vi "Measurement UI.vi"() -> ()   [LabVIEW 2022 SP3, in "Single Tone No Gen_Class D Amplifier_UI.lvlib"]
uses:
  Single Tone No Gen_Class D Amplifier_UI.lvlib
  shared/controls/units - snr.ctl
  shared/controls/units - ratio.ctl
  shared/ui/controls/view.ctl
  shared/controls/acquisition type.ctl
  UI State.ctl
  <vilib>/Utility/miscctls.llb/LVBoundsTypeDef.ctl
  <vilib>/Utility/miscctls.llb/LVPoint32TypeDef.ctl
  <vilib>/Utility/miscctls.llb/LVPointTypeDef.ctl
  shared/ui/UI Helpers.lvlib
  shared/audio popup ui/Audio Popup UI.lvlib
  shared/controls/audio controls.lvlib
panel:
  in  "view legend":T1
  out "time domain":waveform(dbl)[](graph)
  out "frequency domain":cluster{"x0":dbl, "dx":dbl, "magnitude":dbl[]}[](graph)
  out "meas table":string[][](table)
  in  "input configuration file":string
  out "output power (W)":dbl[](array[numeric])
  out "SFDR (dBc)":dbl[](array[numeric])
  out "gain":dbl[](array[numeric])
  out "dynamic range (dB)":dbl[](array[numeric])
  out "THD":dbl[](array[numeric])
  out "THD+N":dbl[](array[numeric])
  out "SNR":dbl[](array[numeric])
  out "phase (deg)":dbl[](array[numeric])
  out "amplitude (dBFS)":dbl[](array[numeric])
  out "amplitude (Vrms)":dbl[](array[numeric])
  out "frequency (Hz)":dbl[](array[numeric])
  out "channel names":string[](array[string])
  in  "Configuration tab":enum32{"Acquisition", "Measurement", "Units"}(tab)
  in  "digital channel list":string caption="Digital audio channel"
  in  "configure input":bool
  in  "acquisition type":T2 caption="Input Type"
  in  "Acquisition channel":tag
  in  "min measurement time (s)":dbl=0.1 caption="Minimum measurement time" format="%#_6ps"
  in  "min measurement cycles":u32 caption="Minimum measurement cycles"
  in  "min settling time (s)":dbl=0.1 caption="Minimum settling time" format="%#_6ps"
  in  "min settling cycles":u32 caption="Minimum settling cycles"
  in  "expected amplitude (Vpk)":dbl=1000.0 caption="Expected amplitude" format="%#_6f Vpk"
  in  "lowpass filter":T3(ring) caption="Lowpass filter"
  in  "highpass filter":enum32{"DC", "AC"}(ring) caption="Highpass filter"
  in  "band start":dbl=20.0 caption="Band start" format="%#_6pHz"
  in  "band stop":dbl=20000.0 caption="Band stop" format="%#_6pHz"
  in  "weighting filter":T4(ring)=enum."A-weighting" caption="Weighting filter"
  in  "load impedance":dbl=4.0 caption="Load impedance" format="%#_6p Ohms"
  in  "amplitude reference (Vpk-pk)":dbl=15.0 caption="Amplitude reference" format="%.3p Vpk-pk"
  in  "expected signal frequency":dbl=1000.0 caption="Expected frequency" format="%#_6pHz"
  in  "gain units":T5 caption="Gain"
  in  "THD units":T5 caption="THD"
  in  "THD+N units":T5 caption="THD+N"
  in  "SNR units":T6 caption="SNR"
  out "fft - data":dbl[](array[numeric])
  out "fft - df":dbl
  out "fft - f0":dbl
  out "wfm - data":dbl[](array[numeric])
  out "wfm - dt":dbl
  out "wfm - t0":dbl
  in  "analog input channel":string="PXI1Slot4/ai0"
  # "hidden controls - used to sync with MeasLink"
  # "hidden indicators"
  # "Acquisition"
  # "Filters"
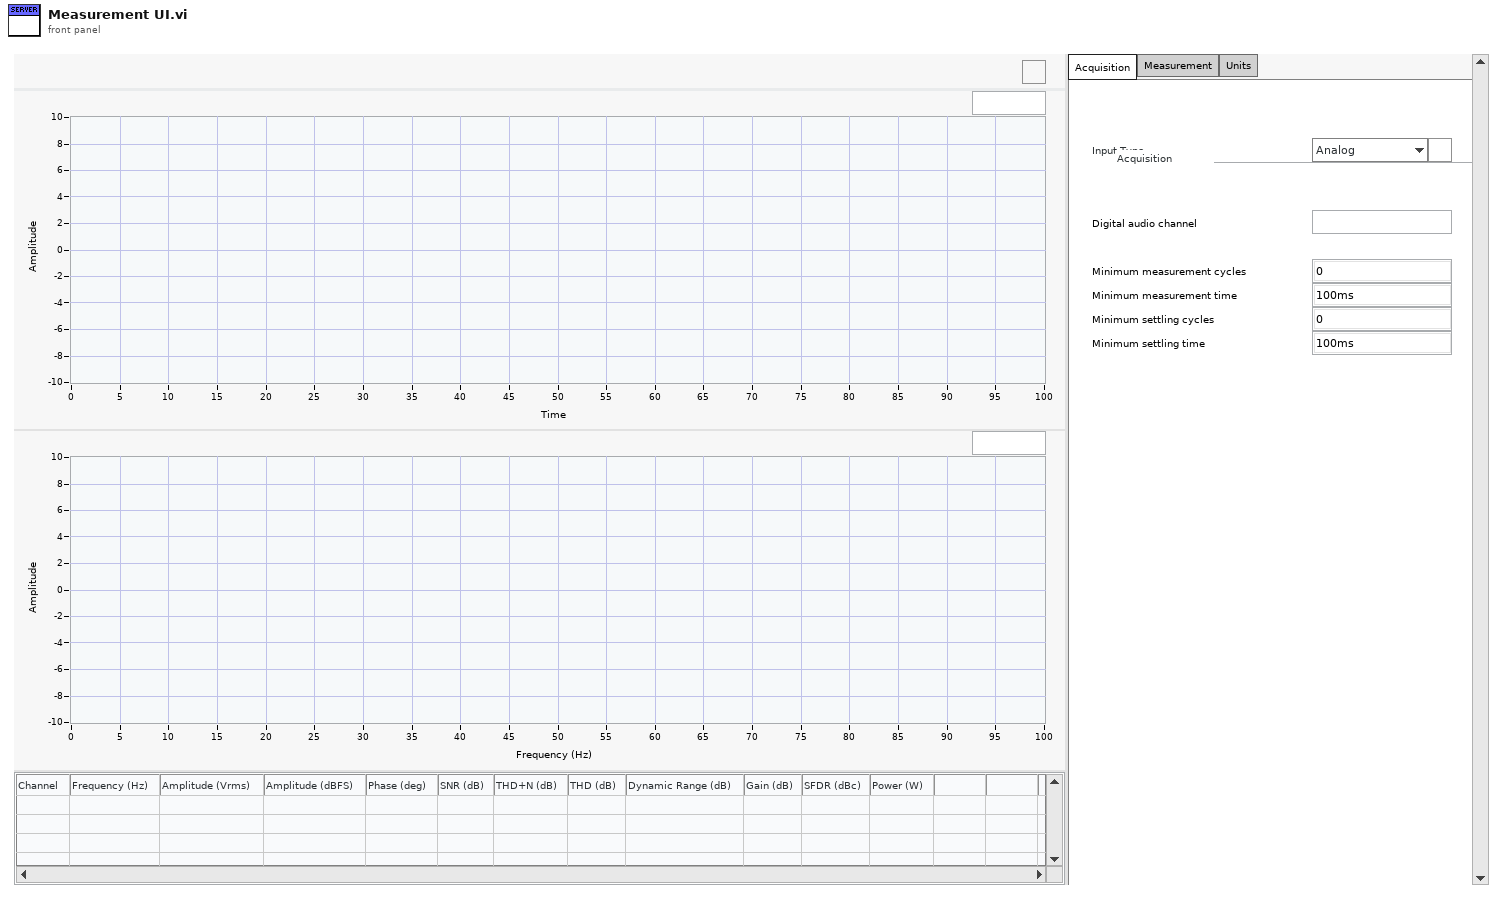
[diagram p1: front panel]
types:
  T1 = typedef "UI Helpers.lvlib/view.ctl" = bool
  T2 = typedef "acquisition type.ctl" = enum32{"Analog", "Digital Serial"}
  T3 = enum32{"No filter", "AES17 20kHz", "AES17 40kHz"}
  T4 = enum32{"Linear", "A-weighting", "B-weighting", "C-weighting"}
  T5 = typedef "audio controls.lvlib/units - ratio.ctl" = enum32{"dB", "%", "x/y"}
  T6 = typedef "audio controls.lvlib/units - snr.ctl" = enum32{"dB", "x/y"}
  T7 = typedef "Single Tone No Gen_Class D Amplifier_UI.lvlib/UI State.ctl" = cluster{"Graph Size":T8, "Legend Visible":bool, "Mouse Coords":T9, "Show All Plots":bool, "digital serial cfg file":path, "analog cfg file":path, "PostUI event occurred":bool}
  T8 = typedef "LVBoundsTypeDef.ctl" = cluster{"Width":u32, "Height":u32}
  T9 = typedef "LVPoint32TypeDef.ctl" = cluster{"Horizontal":i32, "Vertical":i32}
  T10 = typedef "LVPointTypeDef.ctl" = cluster{"Horizontal":i16, "Vertical":i16}
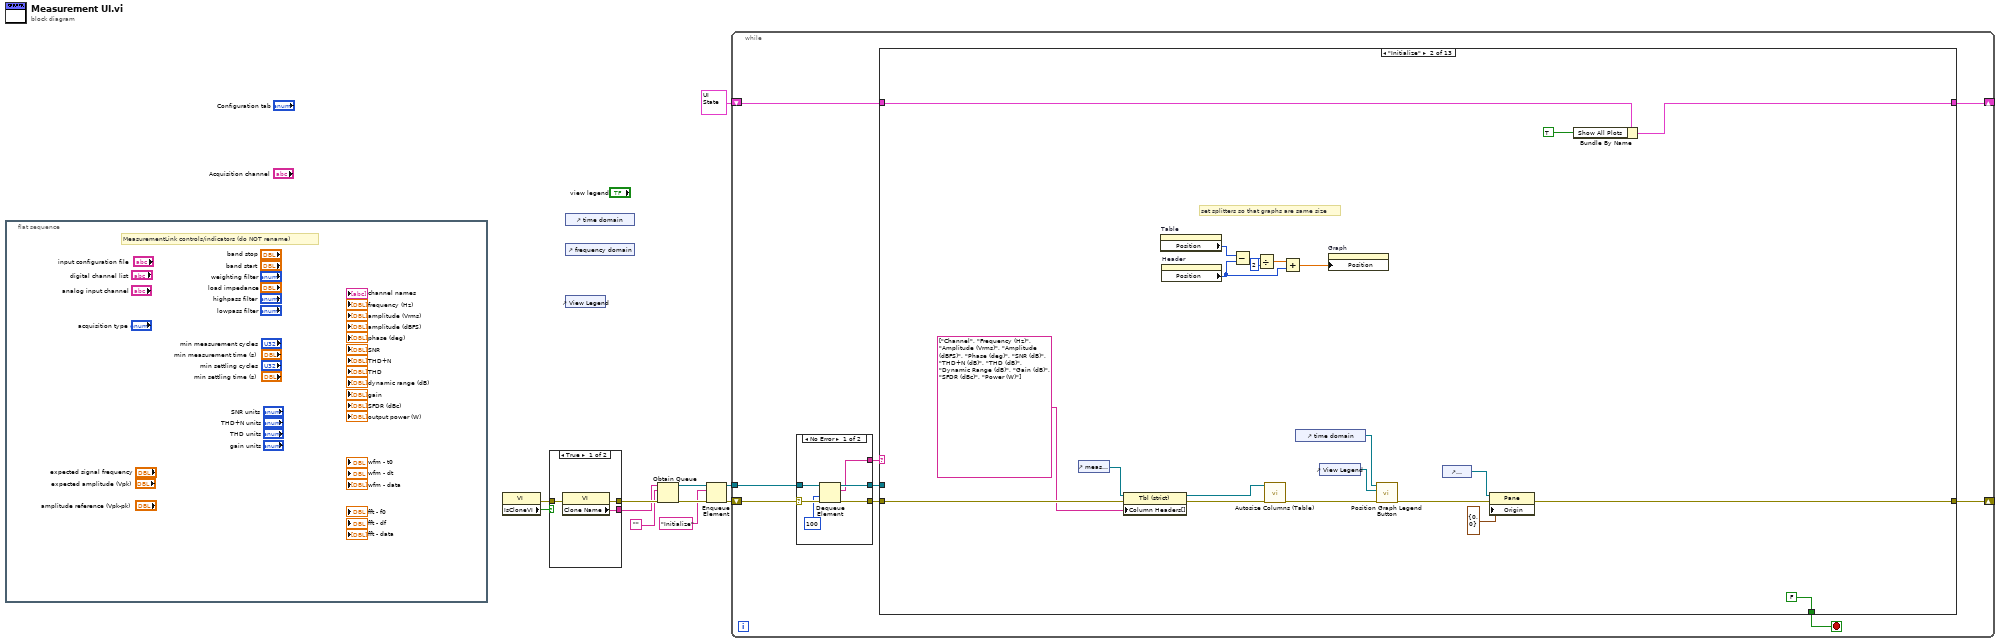
[diagram p0: block diagram]
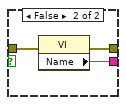
[diagram p2: hidden frame]
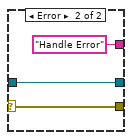
[diagram p3: hidden frame]
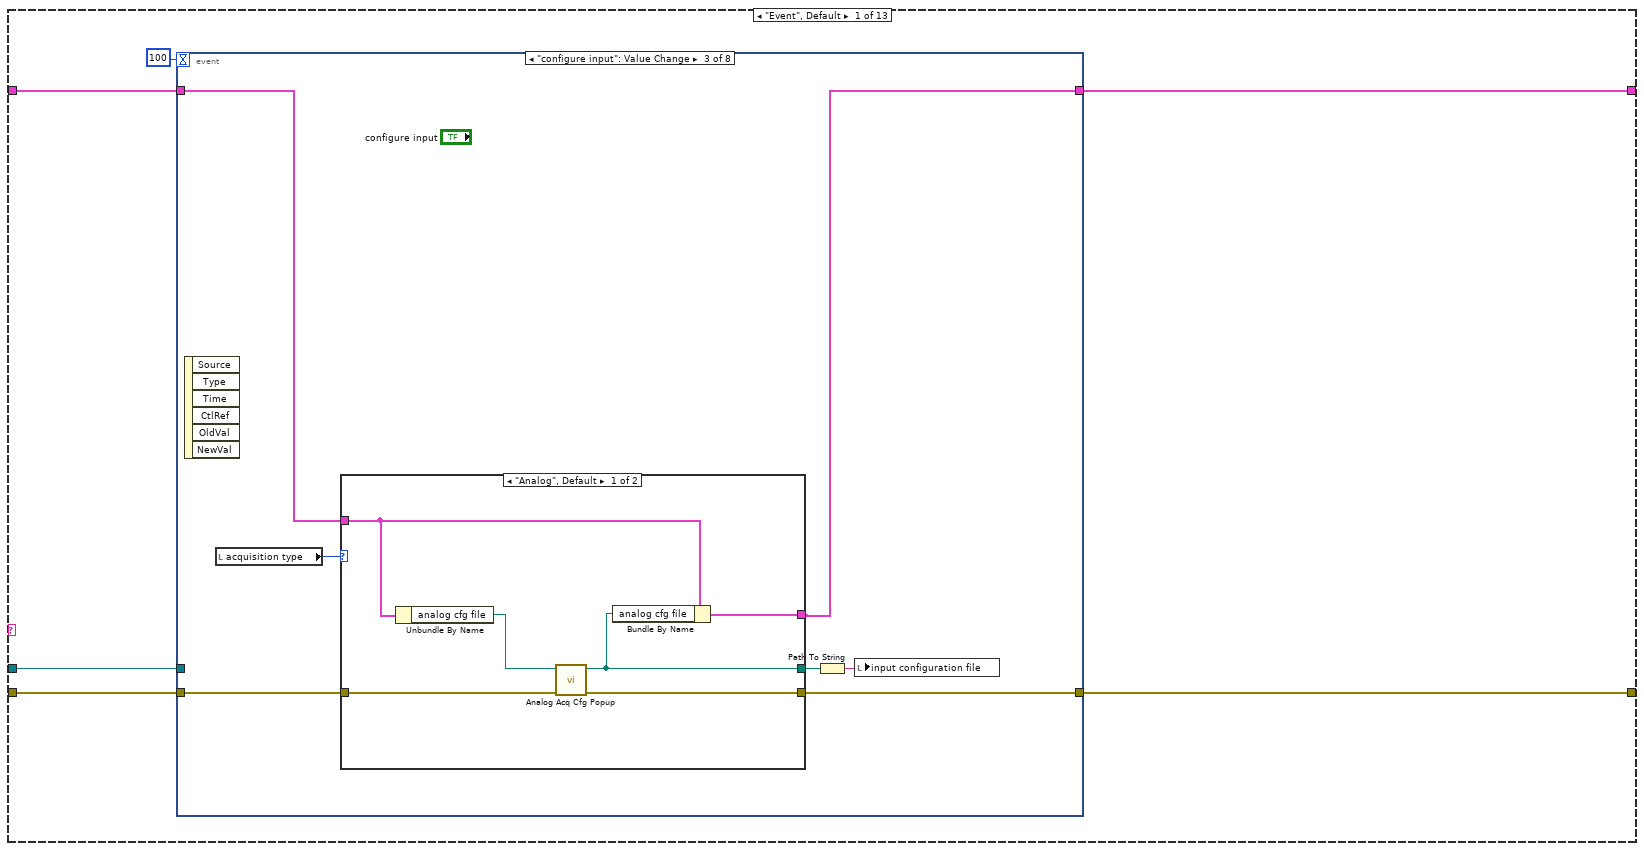
[diagram p4: hidden frame]
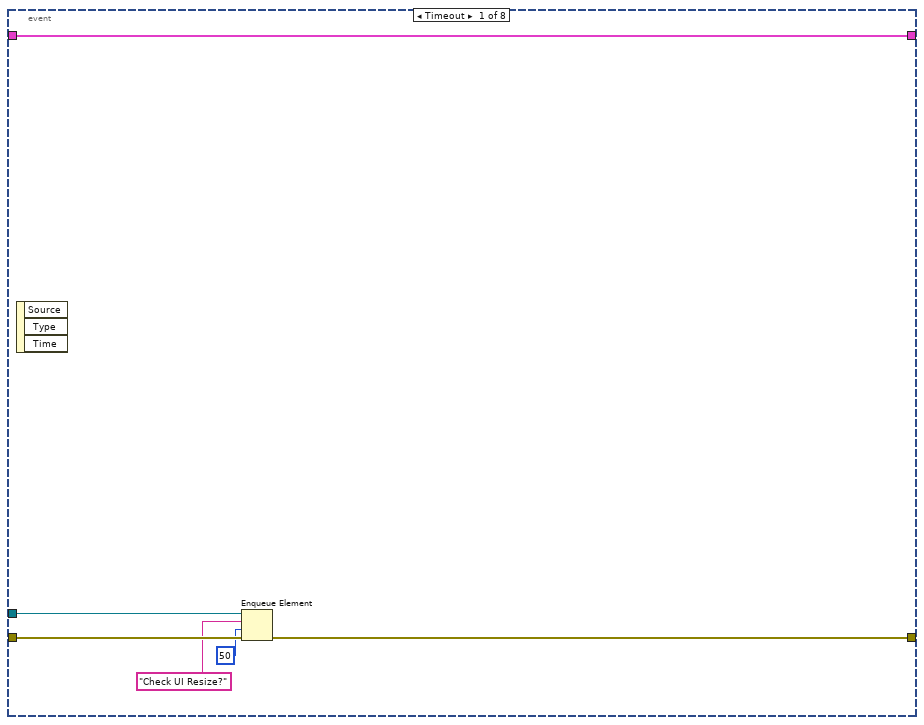
[diagram p5: hidden frame]
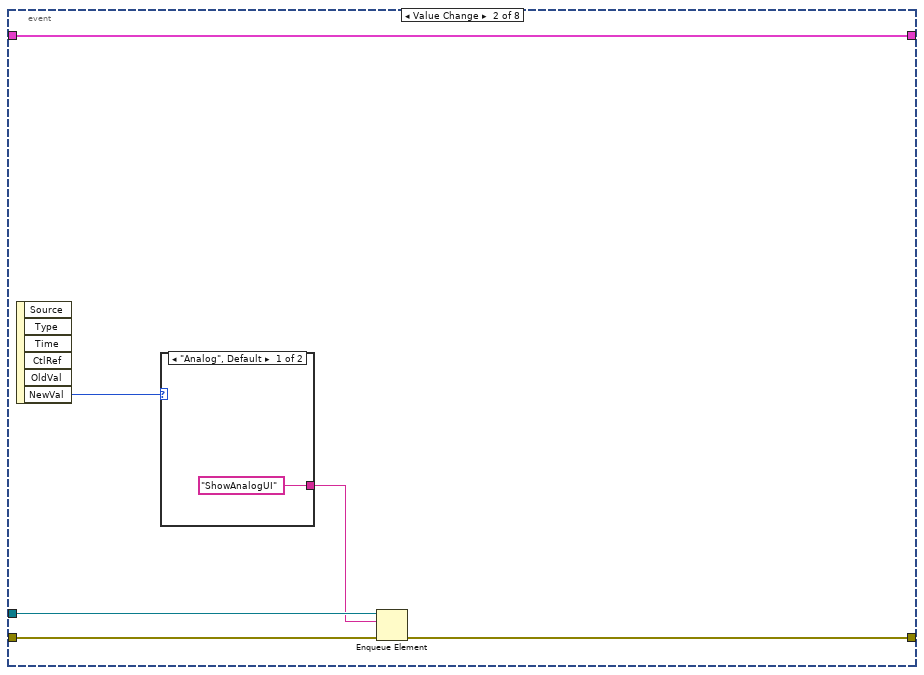
[diagram p6: hidden frame]
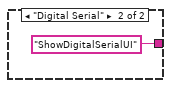
[diagram p7: hidden frame]
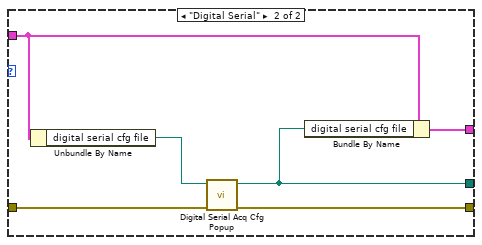
[diagram p8: hidden frame]
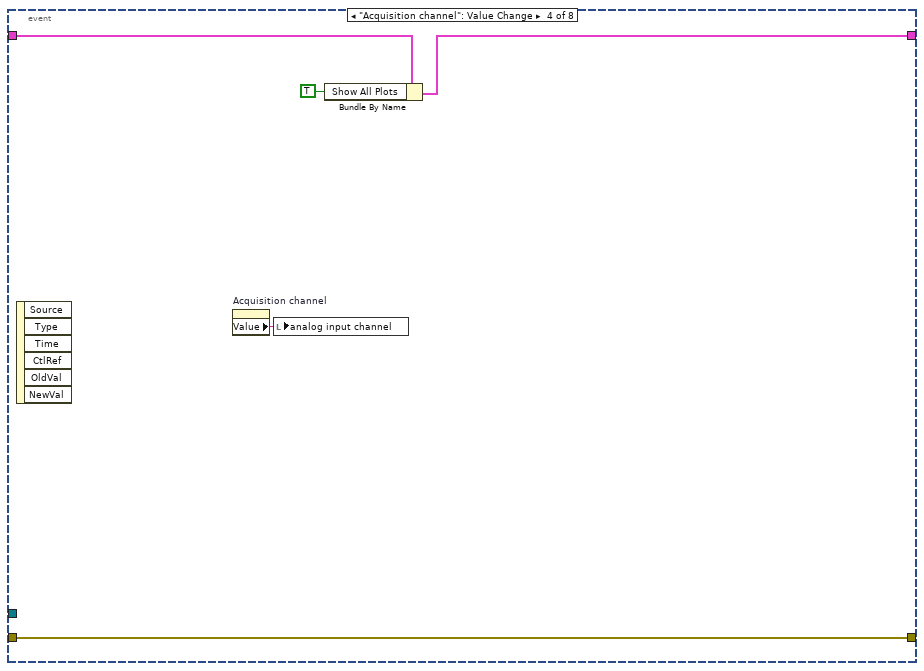
[diagram p9: hidden frame]
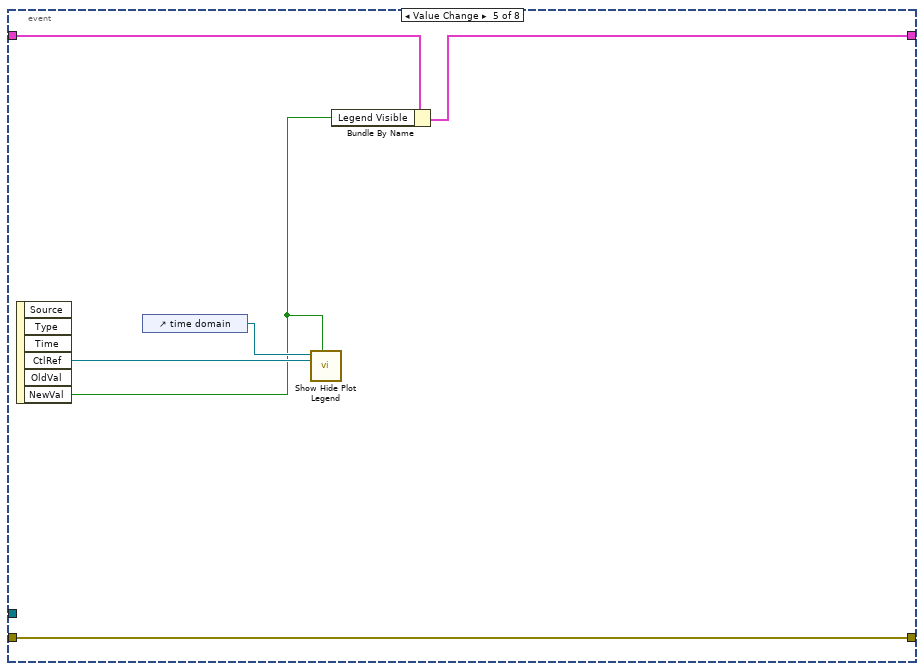
[diagram p10: hidden frame]
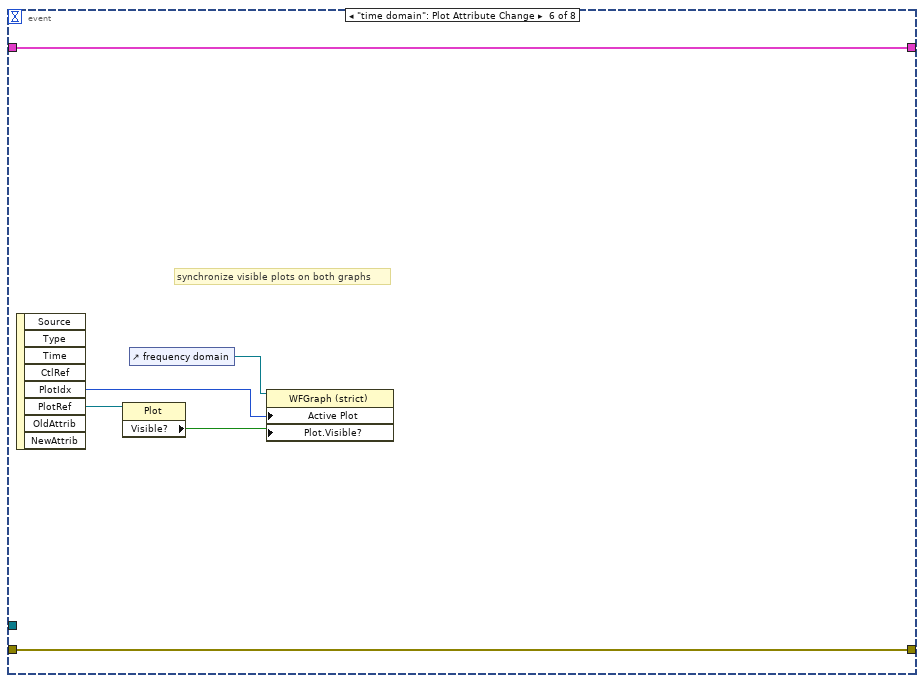
[diagram p11: hidden frame]
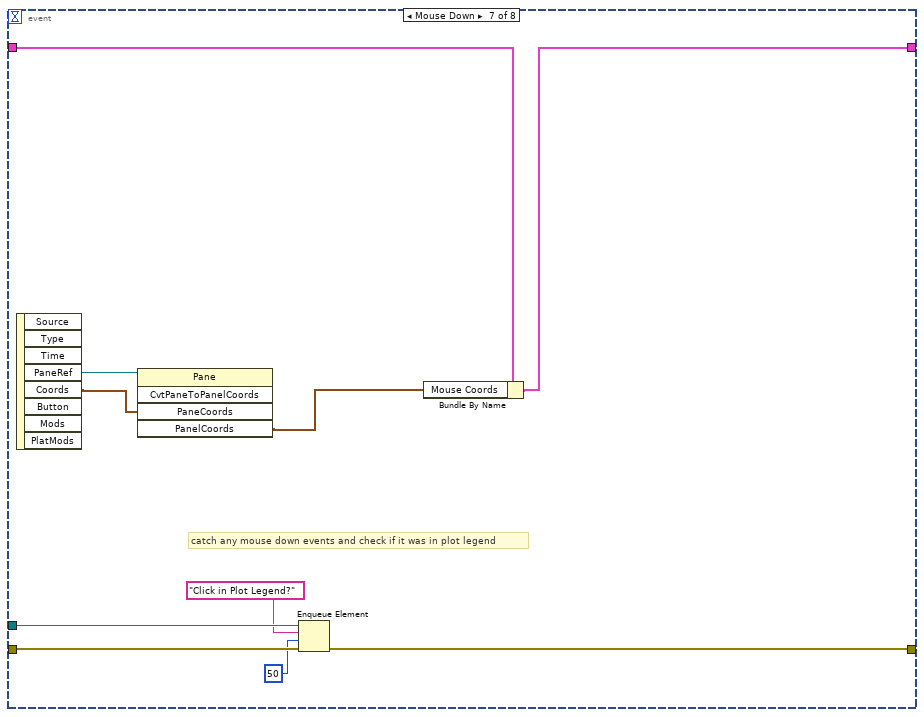
[diagram p12: hidden frame]
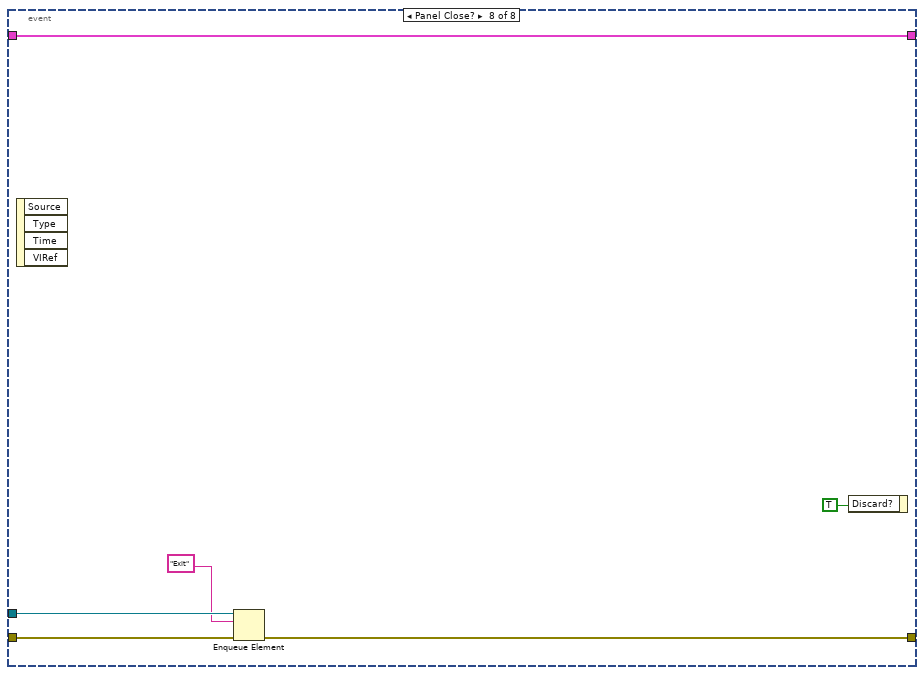
[diagram p13: hidden frame]
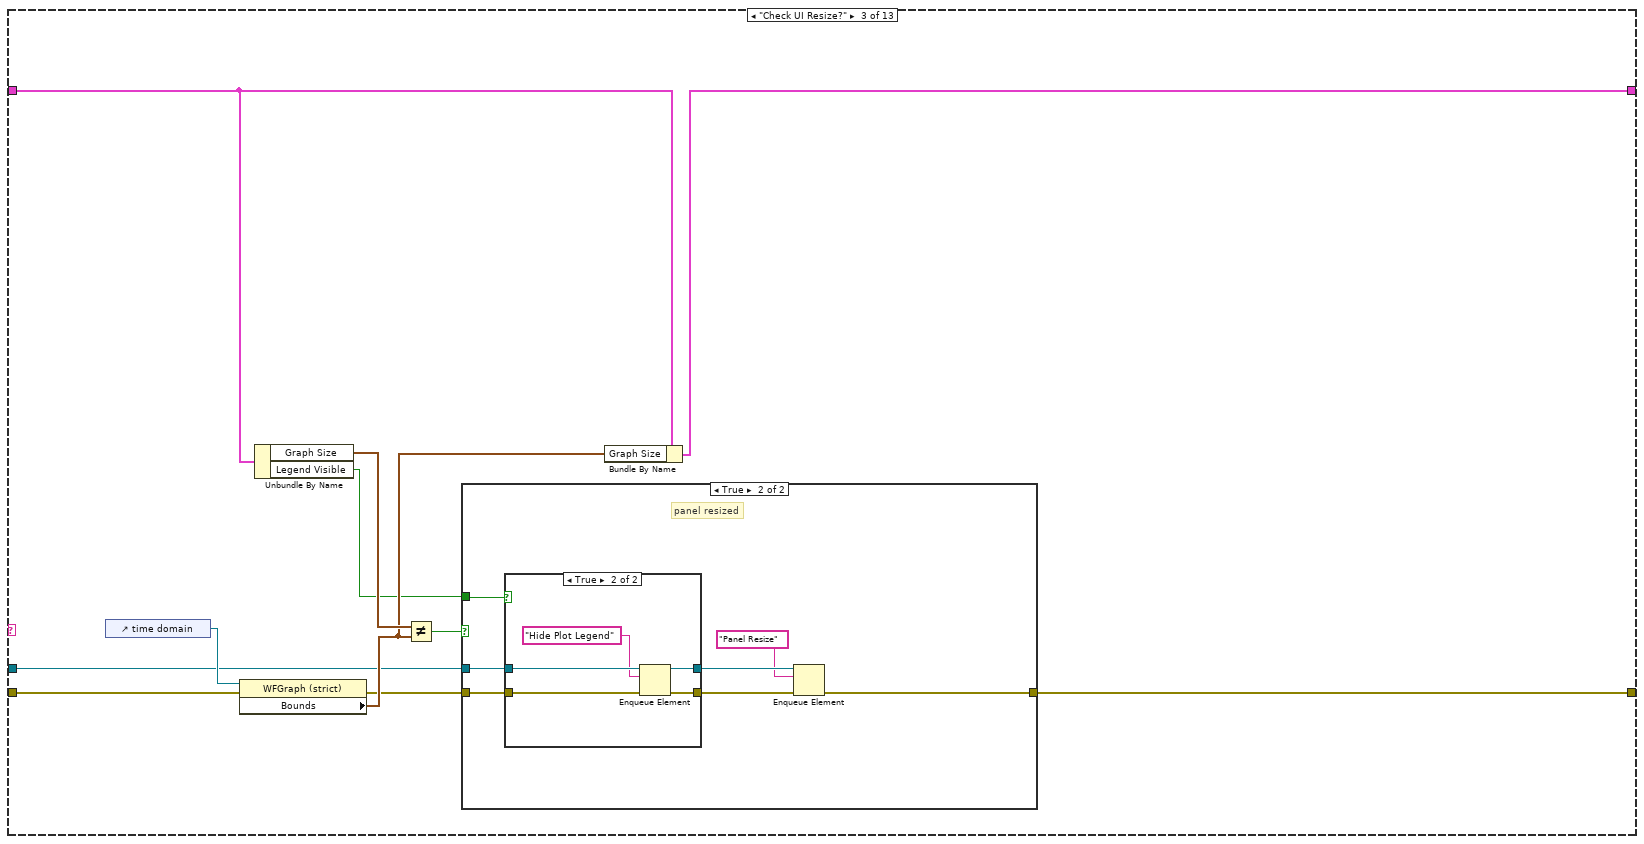
[diagram p14: hidden frame]
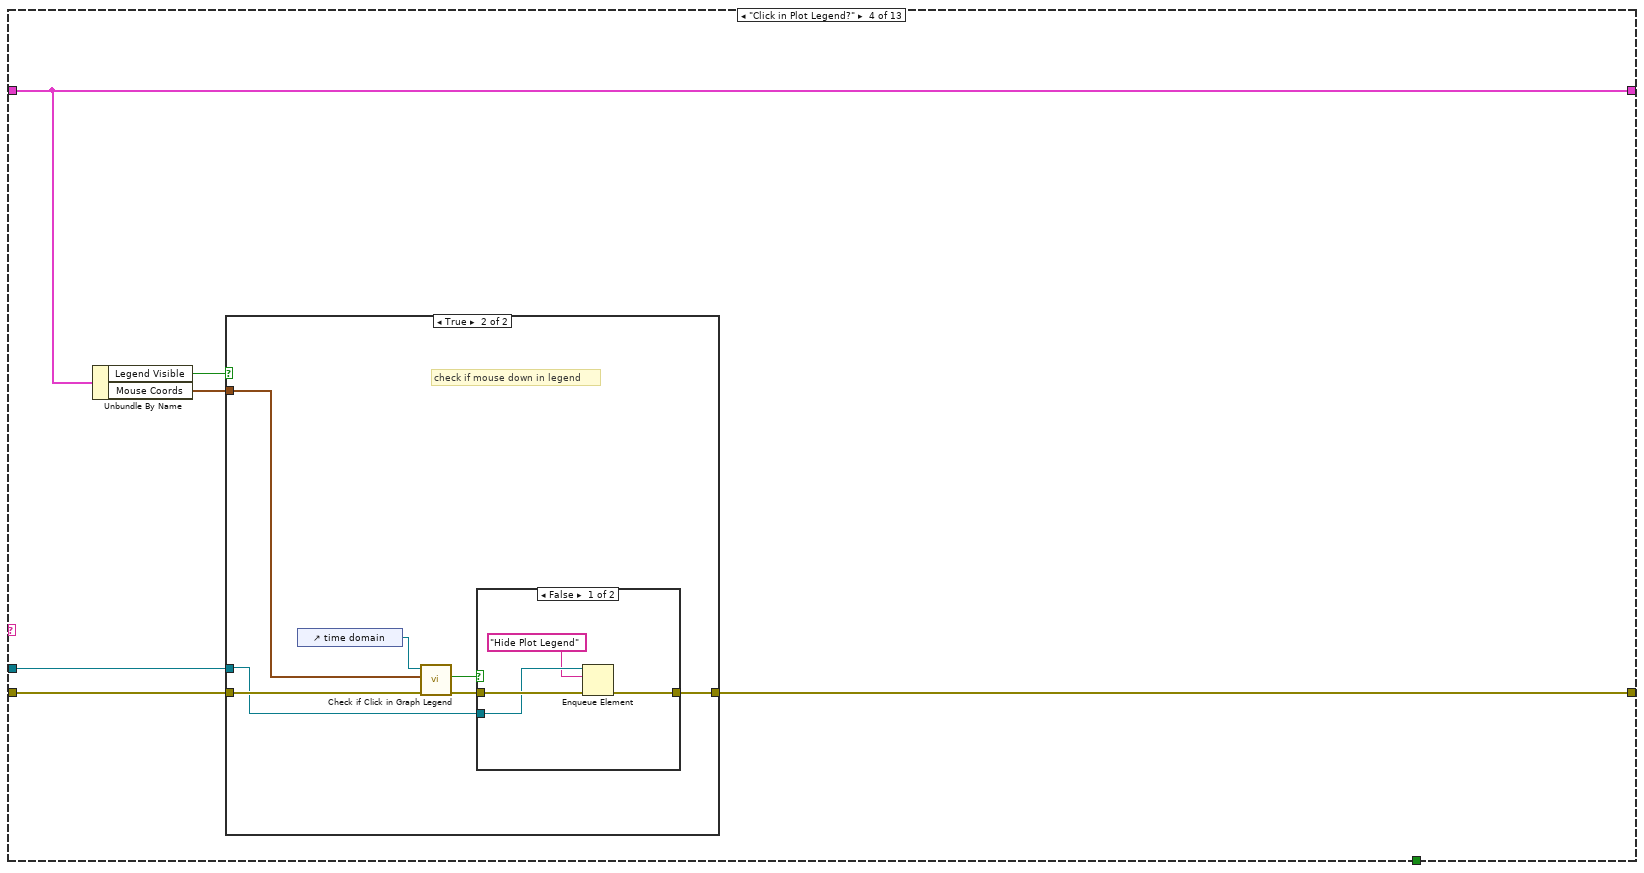
[diagram p17: hidden frame]
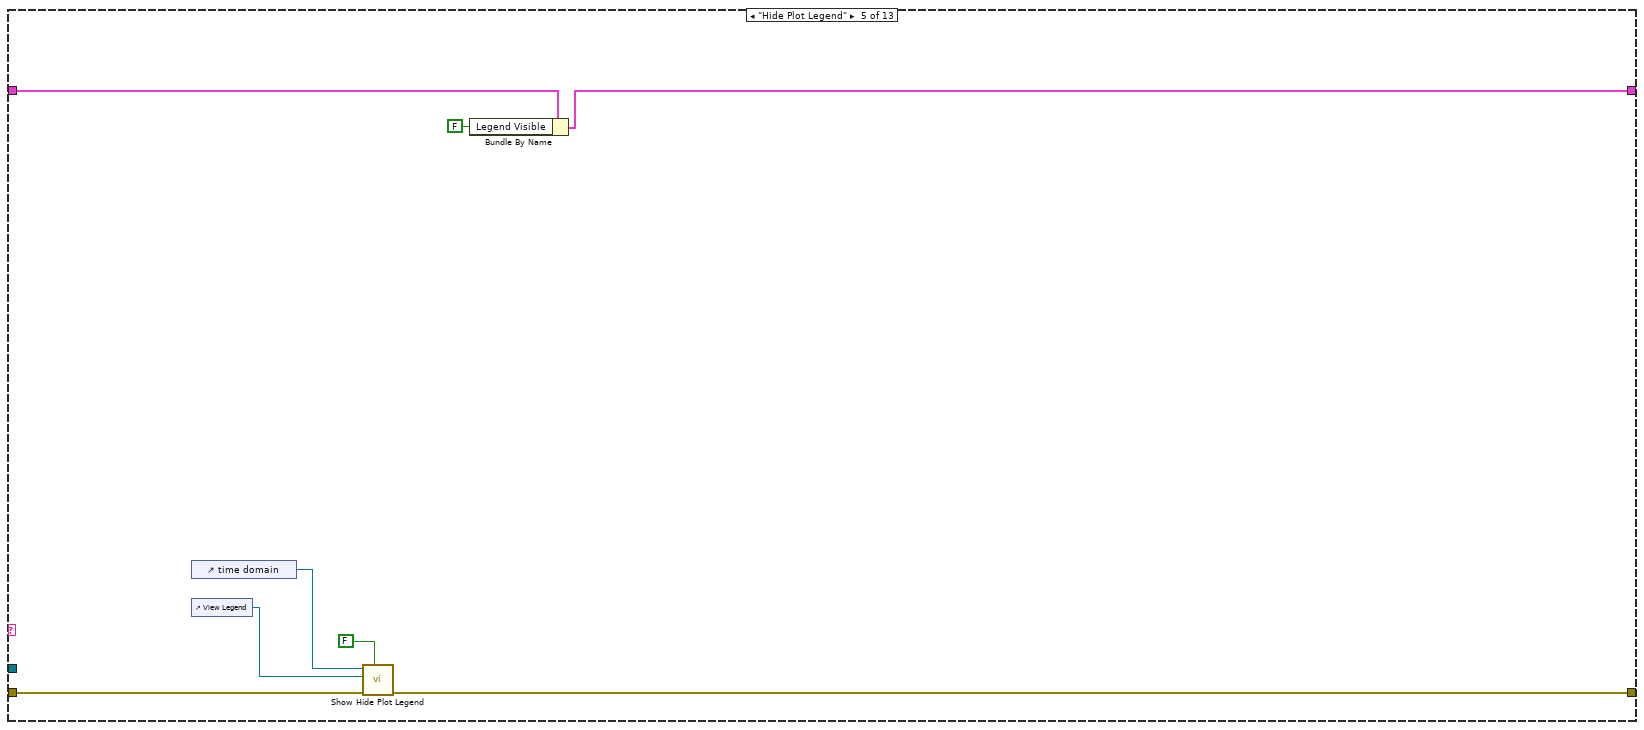
[diagram p20: hidden frame]
diagram:
  n1 = flat-sequence {
    frame #0 {
      # "MeasurementLink controls/indicators (do NOT rename)"
    }
  }
  n2 = property class="VI"() -> (error out=w2:errorcluster, "IsCloneVI"=w3:bool)  [unwired: 2 in, 1 out]
  n3 = case shown="True" w3 {
    tunnel: [w14 w17] -> w11
    tunnel: [w13 w16] -> w10
    tunnel: w2 -> [w12 w15]
    frame True {
      n4 = property class="VI"(error in=w12) -> (error out=w14:errorcluster, "Clone Name"=w13:string)  [unwired: 1 in, 1 out]
    }
    frame False {
      n5 = property class="VI"(error in=w15) -> (error out=w17:errorcluster, "Name"=w16:string)  [unwired: 1 in, 1 out]
    }
  }
  n6 = control-ref of="time domain"() -> ()  [unwired: 1 out]
  n7 = control-ref of="frequency domain"() -> ()  [unwired: 1 out]
  n8 = control-ref of="View Legend"() -> ()  [unwired: 1 out]
  n9 = Obtain Queue(name (unnamed)=w10, element data type="", error in (no error)=w11) -> (queue out=w7:refnum<queue>, error out=w9:errorcluster)  [unwired: 2 in, 1 out]
  n10 = Enqueue Element(queue=w7, element="Initialize", error in (no error)=w9) -> (queue out=w6:refnum<queue>, error out=w8:errorcluster)  [unwired: 1 in, 1 out]
  n11 = while {
    shift-right: [w21] -> _
    shift-left: w8 -> [w26]
    tunnel: w6 -> [w24]
    shift-right: [w19] -> _
    shift-left: T7 {"Graph Size"={"Width"=0, "Height"=0}, "Legend Visible"=FALSE, "Mouse Coords"={"Horizontal"=0, "Vertical"=0}, "Show All Plots"=FALSE, "digital serial cfg file"=path "", "analog cfg file"=path "", "PostUI event occurred"=FALSE} ("ui state") -> [w18]
    stop <- w20 stop-if-true
    n12 = case shown="No Error" w26 {
      selector: w26 -> [w32 w35]
      tunnel: [w31 w35] -> w25
      tunnel: w24 -> [w30 w34]
      tunnel: [w29 w34] -> w23
      tunnel: [w28 "Handle Error"] -> w22
      frame No Error {
        n13 = Dequeue Element(queue=w30, timeout in ms (-1)=100, error in (no error)=w32) -> (queue out=w29:refnum<queue>, element=w28:string, error out=w31:errorcluster)  [unwired: 1 out]
      }
      frame Error {
      }
    }
    n14 = case shown="\"Initialize\"" w22 {
      tunnel: w25 -> [w40 w125 w139 w157 w179 w184 w195 w247 w259 w380 w386 w397 w399]
      tunnel: w23 -> [w38 _ w130 w158 _ _ w191 _ _ _ _ w395 _]
      tunnel: [w41 w109 w132 w156 w178 w183 w192 w247 w263 w380 w386 w392 w399] -> w21
      tunnel: [_ FALSE _ _ _ _ _ _ _ _ _ TRUE _] -> w20
      tunnel: [w36 w114 w135 w161 w180 w187 w188 w239 w260 w383 w389 w390 w398] -> w19
      tunnel: w18 -> [w37 w108 w136 w161 w181 w187 w190 w240 w260 w383 w389 w390 w398]
      frame "Event", Default {
        n15 = event shown="[2] \"configure input\": Value Change" {
          selector: _ -> [_ _ _ _ _ _ _ _]
          dyn-events: _ -> [_ _ _ _ _ _ _ _]
          timeout: 100 -> [_ _ _ _ _ _ _ _]
          tunnel: [w44 w49 w58 w78 w82 w86 w99 w105] -> w41
          tunnel: w40 -> [w47 w51 w61 w78 w82 w86 w100 w106]
          tunnel: w38 -> [w46 w50 _ _ _ _ w101 w104]
          tunnel: w37 -> [w43 w53 w60 w77 w84 w87 w96 w102]
          tunnel: [w43 w53 w59 w76 w83 w87 w95 w102] -> w36
          event Timeout {
            n16 = event-data() -> ()  [unwired: 1 in, 3 out]
            n17 = Enqueue Element(queue=w46, element="Check UI Resize?", timeout in ms (-1)=50, error in (no error)=w47) -> (error out=w44:errorcluster)  [unwired: 2 out]
          }
          event Value Change {
            n18 = event-data() -> ("NewVal"=w52:T2)  [unwired: 1 in, 5 out]
            n19 = case shown="\"Analog\", Default" w52 {
              tunnel: ["ShowAnalogUI" ("element") "ShowDigitalSerialUI" ("element")] -> w48
              frame "Analog", Default {
              }
              frame "Digital Serial" {
              }
            }
            n20 = Enqueue Element(queue=w50, element=w48, error in (no error)=w51) -> (error out=w49:errorcluster)  [unwired: 1 in, 2 out]
          }
          event "configure input": Value Change {
            n21 = event-data() -> ()  [unwired: 1 in, 6 out]
            n22 = local read "acquisition type"() -> (w62:T2)
            n23 = case shown="\"Analog\", Default" w62 {
              tunnel: w61 -> [w68 w74]
              tunnel: [w67 w69] -> w58
              tunnel: [w65 w71] -> w57
              tunnel: w60 -> [w64 w72]
              tunnel: [w63 w70] -> w59
              frame "Analog", Default {
                n24 = Unbundle By Name(w64) -> ("analog cfg file"=w66:path)
                n25 = call "Analog Acq Cfg Popup.vi"("error in (no error)"=w68, "config file in"=w66) -> ("error out"=w67:errorcluster, "config file out"=w65:path)  [unwired: 8 in]
                n26 = Bundle By Name(cluster=w64, "analog cfg file"=w65) -> (w63:T7)
              }
              frame "Digital Serial" {
                n27 = Unbundle By Name(w72) -> ("digital serial cfg file"=w73:path)
                n28 = call "Digital Serial Acq Cfg Popup.vi"("error in (no error)"=w74, "config file in"=w73) -> ("error out"=w69:errorcluster, "config file out"=w71:path)  [unwired: 7 in, 1 out]
                n29 = Bundle By Name(cluster=w72, "digital serial cfg file"=w71) -> (w70:T7)
              }
            }
            n30 = Path To String(path=w57) -> (string=w56:string)
            n31 = local write "input configuration file"(w56) -> ()
          }
          event "Acquisition channel": Value Change {
            n32 = event-data() -> ()  [unwired: 1 in, 6 out]
            n33 = property on="Acquisition channel" class="DAQmxName"() -> ("Value"=w79:string)  [unwired: 2 in, 2 out]
            n34 = local write "analog input channel"(w79) -> ()
            n35 = Bundle By Name(cluster=w77, "Show All Plots"=TRUE) -> (w76:T7)
          }
          event Value Change {
            n36 = event-data() -> ("CtlRef"=w81:refnum<vi>, "NewVal"=w80:T1)  [unwired: 1 in, 4 out]
            n37 = control-ref of="time domain"() -> (w85:refnum<vi>)
            n38 = call "Show Hide Plot Legend.vi"("show"=w80, "view reference"=w81, "graph reference"=w85) -> ()  [unwired: 8 in, 1 out]
            n39 = Bundle By Name(cluster=w84, "Legend Visible"=w80) -> (w83:T7)
          }
          event "time domain": Plot Attribute Change {
            # "synchronize visible plots on both graphs"
            n40 = event-data() -> ("PlotIdx"=w89:i32, "PlotRef"=w90:refnum<vi>)  [unwired: 1 in, 6 out]
            n41 = property class="Plot"(reference=w90) -> ("Visible?"=w91:bool)  [unwired: 1 in, 2 out]
            n42 = control-ref of="frequency domain"() -> (w88:refnum<vi>)
            n43 = property on="Property Node" class="WFGraph (strict)"(reference=w88, "Active Plot"=w89, "Plot.Visible?"=w91) -> ()  [unwired: 1 in, 2 out]
          }
          event Mouse Down {
            # "catch any mouse down events and check if it was in plot legend"
            n44 = event-data() -> ("PaneRef"=w94:refnum<vi>, "Coords"=w93:T9)  [unwired: 1 in, 6 out]
            n45 = invoke class="Pane" method="CvtPaneToPanelCoords"(reference=w94, "PaneCoords"=w93) -> ("PanelCoords"=w92:T10)  [unwired: 3 in, 4 out]
            n46 = Enqueue Element(queue=w101, element="Click in Plot Legend?", timeout in ms (-1)=50, error in (no error)=w100) -> (error out=w99:errorcluster)  [unwired: 2 out]
            n47 = Bundle By Name(cluster=w96, "Mouse Coords"=w92) -> (w95:T7)
          }
          event Panel Close? {
            n48 = event-data() -> ()  [unwired: 1 in, 4 out]
            n49 = Enqueue Element(queue=w104, element="Exit", error in (no error)=w106) -> (error out=w105:errorcluster)  [unwired: 1 in, 2 out]
            n50 = event-data("Discard?"=TRUE) -> ()  [unwired: 1 in, 1 out]
          }
        }
      }
      frame "Initialize" {
        # "set splitters so that graphs are same size"
        n51 = control-ref of="meas table"() -> (w123:refnum<vi>)
        n52 = property class="Tbl (strict)"(reference=w123, error in=w125, "Column Headers[]"=string[] ["Channel", "Frequency (Hz)", "Amplitude (Vrms)", "Amplitude (dBFS)", "Phase (deg)", "SNR (dB)", "THD+N (dB)", "THD (dB)", "Dynamic Range (dB)", "Gain (dB)", "SFDR (dBc)", "Power (W)"] ("Column Header Strings[]")) -> (reference out=w122:refnum<vi>, error out=w124:errorcluster)
        n53 = property on="Table" class="Splitter"() -> ("Position"=w120:i32)  [unwired: 2 in, 2 out]
        n54 = property on="Header" class="Splitter"() -> ("Position"=w116:i32)  [unwired: 2 in, 2 out]
        n55 = Subtract(x=w120, y=w116) -> (x-y=w119:i32)
        n56 = Divide(x=w119, y=2) -> (x/y=w117:dbl)
        n57 = call "Autosize Columns (Table).vi"("error in (no error)"=w124, "table"=w122) -> ("error out"=w126:errorcluster)  [unwired: 9 in]
        n58 = Add(x=w117, y=w116) -> (x+y=w115:dbl)
        n59 = control-ref of="time domain"() -> (w128:refnum<vi>)
        n60 = control-ref of="View Legend"() -> (w127:refnum<vi>)
        n61 = property on="Graph" class="Splitter"("Position"=w115) -> ()  [unwired: 2 in, 2 out]
        n62 = call "Position Graph Legend Button.vi"("error in (no error)"=w126, "view legend"=w127, "graph"=w128) -> ("error out"=w112:errorcluster)  [unwired: 8 in]
        n63 = control-ref of="Configuration"() -> (w111:refnum<vi>)
        n64 = property class="Pane"(reference=w111, error in=w112, "Origin"=T10 {"Horizontal"=0, "Vertical"=0}) -> (error out=w109:errorcluster)  [unwired: 1 out]
        n65 = Bundle By Name(cluster=w108, "Show All Plots"=TRUE ("Init Graph Plot Legend")) -> (w114:T7)
      }
      frame "Check UI Resize?" {
        n66 = control-ref of="time domain"() -> (w140:refnum<vi>)
        n67 = property on="Property Node" class="WFGraph (strict)"(reference=w140, error in=w139) -> (error out=w133:errorcluster, "Bounds"=w137:T8)  [unwired: 1 out]
        n68 = Unbundle By Name(w136) -> ("Graph Size"=w138:T8, "Legend Visible"=w131:bool)
        n69 = Not Equal?(x=w138, y=w137) -> (x != y?=w134:bool)
        n70 = case shown="True" w134 {
          tunnel: w133 -> [w141 w148]
          tunnel: [w141 w143] -> w132
          tunnel: w131 -> [_ w146]
          tunnel: w130 -> [_ w147]
          frame False {
            # "no resize"
          }
          frame True {
            # "panel resized"
            n71 = case shown="True" w146 {
              tunnel: w148 -> [w150 w155]
              tunnel: [w150 w154] -> w145
              tunnel: w147 -> [w149 w153]
              tunnel: [w149 w151] -> w144
              frame False {
              }
              frame True {
                n72 = Enqueue Element(queue=w153, element="Hide Plot Legend", error in (no error)=w155) -> (queue out=w151:refnum<queue>, error out=w154:errorcluster)  [unwired: 1 in, 1 out]
              }
            }
            n73 = Enqueue Element(queue=w144, element="Panel Resize", error in (no error)=w145) -> (error out=w143:errorcluster)  [unwired: 1 in, 2 out]
          }
        }
        n74 = Bundle By Name(cluster=w136, "Graph Size"=w137) -> (w135:T7)
      }
      frame "Click in Plot Legend?" {
        n75 = Unbundle By Name(w161) -> ("Legend Visible"=w160:bool, "Mouse Coords"=w159:T9)
        n76 = case shown="True" w160 {
          tunnel: w159 -> [_ w167]
          tunnel: w158 -> [_ w164]
          tunnel: w157 -> [w162 w169]
          tunnel: [w162 w163] -> w156
          frame False {
            # "legend not visible; do nothing"
          }
          frame True {
            # "check if mouse down in legend"
            n77 = control-ref of="time domain"() -> (w168:refnum<vi>)
            n78 = call "Check if Click in Graph Legend.vi"("error in (no error)"=w169, "Mouse Coords"=w167, "WaveformGraph"=w168) -> ("error out"=w165:errorcluster, "click in legend?"=w166:bool)  [unwired: 7 in]
            n79 = case shown="False" w166 {
              tunnel: w165 -> [w173 w174]
              tunnel: w164 -> [w172 _]
              tunnel: [w171 w174] -> w163
              frame False {
                n80 = Enqueue Element(queue=w172, element="Hide Plot Legend", error in (no error)=w173) -> (error out=w171:errorcluster)  [unwired: 1 in, 2 out]
              }
              frame True {
                # "inside legend; do nothing"
              }
            }
          }
        }
      }
      frame "Hide Plot Legend" {
        n81 = control-ref of="time domain"() -> (w176:refnum<vi>)
        n82 = control-ref of="View Legend"() -> (w175:refnum<vi>)
        n83 = call "Show Hide Plot Legend.vi"("show"=FALSE, "error in (no error)"=w179, "view reference"=w175, "graph reference"=w176) -> ("error out"=w178:errorcluster)  [unwired: 7 in]
        n84 = Bundle By Name(cluster=w181, "Legend Visible"=FALSE ("legend visible")) -> (w180:T7)
      }
      frame "Panel Resize" {
        n85 = control-ref of="time domain"() -> (w186:refnum<vi>)
        n86 = control-ref of="View Legend"() -> (w185:refnum<vi>)
        n87 = call "Position Graph Legend Button.vi"("error in (no error)"=w184, "view legend"=w185, "graph"=w186) -> ("error out"=w183:errorcluster)  [unwired: 8 in]
      }
      frame "Post UI Update" {
        # "This case will be triggered, after framework updates the User interface with result values."
        n88 = for {
          tunnel: w191 -> [w225]
          shift-right: [w224] -> w193
          shift-left: w195 -> [w226]
          tunnel: string[] ["Update Table", "Update Graphs"] -> [w223] mode=indexing
          n89 = Enqueue Element(queue=w225, element=w223, timeout in ms (-1)=50, error in (no error)=w226) -> (error out=w224:errorcluster)  [unwired: 2 out]
        }
        n90 = Unbundle By Name(w190) -> ("PostUI event occurred"=w189:bool)
        n91 = case shown="False" w189 {
          tunnel: w193 -> [w198 w222]
          tunnel: w191 -> [w205 _]
          tunnel: [w196 w222] -> w192
          tunnel: w190 -> [w204 w221]
          tunnel: [w201 w221] -> w188
          frame False {
            # "do this on first PostUI Event (happens when panel loads)"
            n92 = local read "input configuration file"() -> (w208:string)
            n93 = local read "analog input channel"() -> (w199:string)
            n94 = String To Path(string=w208) -> (path=w200:path)
            n95 = local write "Acquisition channel"(w199) -> ()
            n96 = call "Determine Acquisition Type from File.vi"("cfg file"=w200) -> ("output type"=w206:T2)  [unwired: 9 in, 1 out]
            n97 = local write "acquisition type"(w206) -> ()
            n98 = Bundle By Name(cluster=w204, "PostUI event occurred"=TRUE) -> (w202:T7)
            n99 = case shown="\"Analog\", Default" w206 {
              tunnel: ["ShowAnalogUI" ("element") "ShowDigitalSerialUI" ("element")] -> w207
              tunnel: w202 -> [w213 w219]
              tunnel: [w212 w218] -> w201
              tunnel: w200 -> [w210 w216]
              tunnel: w198 -> [w209 w215]
              tunnel: [w209 w215] -> w197
              frame "Analog", Default {
                n100 = Bundle By Name(cluster=w213, "digital serial cfg file"=path "", "analog cfg file"=w210) -> (w212:T7)
              }
              frame "Digital Serial" {
                n101 = Bundle By Name(cluster=w219, "digital serial cfg file"=w216, "analog cfg file"=path "") -> (w218:T7)
              }
            }
            n102 = Enqueue Element(queue=w205, element=w207, error in (no error)=w197) -> (error out=w196:errorcluster)  [unwired: 1 in, 2 out]
          }
          frame True {
          }
        }
      }
      frame "Update Graphs" {
        # "This case will be triggered, after framework updates the User interface with result values."
        n103 = local read "channel names"() -> (w243:string[])
        n104 = local read "wfm - data"() -> (w238:dbl[])
        n105 = local read "wfm - dt"() -> (w237:dbl)
        n106 = local read "fft - data"() -> (w236:dbl[])
        n107 = local read "fft - df"() -> (w235:dbl)
        n108 = local read "fft - f0"() -> (w234:dbl)
        n109 = call "Array to Wfm (N Ch).vi"("channel names"=w243, "dt"=w237, "array"=w238) -> ("waveforms"=w232:waveform(dbl)[])  [unwired: 8 in]
        "time domain" <- w232
        n110 = call "Array to Spectra (N Ch).vi"("channel names"=w243, "df"=w235, "f0"=w234, "data"=w236) -> ("spectra"=→"frequency domain":cluster{"f0":dbl, "df":dbl, "data":dbl[]}[])  [unwired: 7 in]
        n111 = Unbundle By Name(w240) -> ("Show All Plots"=w228:bool)
        n112 = control-ref of="time domain"() -> (w246:refnum<vi>)
        n113 = control-ref of="frequency domain"() -> (w242:refnum<vi>)
        n114 = Array Size(array=w232) -> (size(s)=w231:i32)
        n115 = Greater Than 0?(x=w231) -> (x > 0?=w230:bool)
        n116 = And(x=w228, y=w230) -> (x .and. y?=w229:bool)
        n117 = case shown="True" w229 {
          tunnel: w246 -> [_ w252]
          tunnel: w243 -> [_ w251]
          tunnel: w242 -> [_ w250]
          tunnel: [w248 FALSE] -> w241
          tunnel: w228 -> [w248 _]
          frame False {
          }
          frame True {
            # "show all graphs the 1st time data is written"
            n118 = for {
              tunnel: w250 -> [w253]
              tunnel: w251 -> [_] mode=indexing
              i -> [w254]
              # "make all plots visible"
              n119 = property class="WFGraph (strict)"(reference=w253, "Active Plot"=w254, "Plot.Visible?"=TRUE ("Plot.Visible")) -> ()  [unwired: 1 in, 2 out]
            }
            n120 = for {
              tunnel: w252 -> [w256]
              tunnel: w251 -> [_] mode=indexing
              i -> [w257]
              # "make all plots visible"
              n121 = property class="WFGraph (strict)"(reference=w256, "Active Plot"=w257, "Plot.Visible?"=TRUE ("Plot.Visible")) -> ()  [unwired: 1 in, 2 out]
            }
          }
        }
        n122 = Array Size(array=w243) -> (size(s)=w245:i32)
        n123 = property class="WFGraph (strict)"(reference=w246, "LegNumRows"=w245, "LegScrollVis"=FALSE ("Legend:Scrollbar Visible")) -> ()  [unwired: 1 in, 2 out]
        n124 = Bundle By Name(cluster=w240, "Show All Plots"=w241) -> (w239:T7)
      }
      frame "Update Table" {
        # "format data for table"
        # "This case will be triggered, after framework updates the User interface with result values."
        n125 = local read "SNR units"() -> (w303:T6)
        n126 = local read "THD+N units"() -> (w315:T5)
        n127 = local read "THD units"() -> (w301:T5)
        n128 = local read "gain units"() -> (w299:T5)
        n129 = case shown="\"x/y\"" w303 {
          tunnel: ["(dB)" "(ratio)"] -> w314
          tunnel: ["%5.1f" ("initial string") "%.1f" ("initial string")] -> w297
          frame "dB", Default {
          }
          frame "x/y" {
          }
        }
        n130 = case shown="\"x/y\"" w315 {
          tunnel: ["(dB)" "(%)" "(ratio)"] -> w317
          tunnel: ["%5.1f" ("initial string") "%.3f" ("initial string") "%.6f" ("initial string")] -> w294
          frame "dB", Default {
          }
          frame "%" {
          }
          frame "x/y" {
          }
        }
        n131 = case shown="\"x/y\"" w301 {
          tunnel: ["(dB)" "(%)" "(ratio)"] -> w302
          tunnel: ["%5.1f" ("initial string") "%.3f" ("initial string") "%.6f" ("initial string")] -> w291
          frame "dB", Default {
          }
          frame "%" {
          }
          frame "x/y" {
          }
        }
        n132 = case shown="\"%\"" w299 {
          tunnel: ["(dB)" "(%)" "(ratio)"] -> w300
          tunnel: ["%5.1f" ("initial string") "%.1f" ("initial string") "%.3f" ("initial string")] -> w281
          frame "dB", Default {
          }
          frame "%" {
          }
          frame "x/y" {
          }
        }
        n133 = Concatenate Strings("SNR " ("string"), w314) -> (w311:string)
        n134 = Concatenate Strings("THD+N " ("string"), w317) -> (w310:string)
        n135 = Concatenate Strings("Gain " ("string"), w300) -> (w308:string)
        n136 = Concatenate Strings("THD " ("string"), w302) -> (w309:string)
        n137 = property on="meas table" class="Tbl (strict)"() -> ("Column Headers[]"=w264:string[])  [unwired: 2 in, 2 out]
        n138 = Replace Array Subset(array=w264, new element #1=w311, index #1=5 ("index"), new element #2=w310, index #2=6 ("index"), new element #3=w309, index #3=7 ("index"), new element #4=w308, index #4=9 ("index")) -> (w312:string[])
        n139 = property on="meas table" class="Tbl (strict)"("Column Headers[]"=w312) -> ()  [unwired: 2 in, 2 out]
        n140 = local read "amplitude (Vrms)"() -> (w276:dbl[])
        n141 = local read "amplitude (dBFS)"() -> (w273:dbl[])
        n142 = local read "frequency (Hz)"() -> (w279:dbl[])
        n143 = local read "phase (deg)"() -> (w269:dbl[])
        n144 = local read "THD+N"() -> (w296:dbl[])
        n145 = local read "THD"() -> (w293:dbl[])
        n146 = local read "SNR"() -> (w298:dbl[])
        n147 = local read "channel names"() -> (w261:string[])
        n148 = for {
          tunnel: [w334] -> w278 mode=indexing
          tunnel: w279 -> [w333] mode=indexing
          tunnel: "%.3f" ("initial string") -> [w332]
          n149 = Format Into String(format string=w332, w333) -> (resulting string=w334:string)  [unwired: 2 in, 1 out]
        }
        n150 = for {
          tunnel: [w331] -> w275 mode=indexing
          tunnel: w276 -> [w330] mode=indexing
          tunnel: "%.3f" ("initial string") -> [w329]
          n151 = Format Into String(format string=w329, w330) -> (resulting string=w331:string)  [unwired: 2 in, 1 out]
        }
        n152 = for {
          tunnel: [w328] -> w272 mode=indexing
          tunnel: w273 -> [w327] mode=indexing
          tunnel: "%.3f" ("initial string") -> [w326]
          n153 = Format Into String(format string=w326, w327) -> (resulting string=w328:string)  [unwired: 2 in, 1 out]
        }
        n154 = for {
          tunnel: [w349] -> w292 mode=indexing
          tunnel: w293 -> [w348] mode=indexing
          tunnel: w291 -> [w347]
          n155 = Format Into String(format string=w347, w348) -> (resulting string=w349:string)  [unwired: 2 in, 1 out]
        }
        n156 = for {
          tunnel: [w355] -> w287 mode=indexing
          tunnel: w298 -> [w354] mode=indexing
          tunnel: w297 -> [w353]
          n157 = Format Into String(format string=w353, w354) -> (resulting string=w355:string)  [unwired: 2 in, 1 out]
        }
        n158 = for {
          tunnel: [w352] -> w295 mode=indexing
          tunnel: w296 -> [w351] mode=indexing
          tunnel: w294 -> [w350]
          n159 = Format Into String(format string=w350, w351) -> (resulting string=w352:string)  [unwired: 2 in, 1 out]
        }
        n160 = for {
          tunnel: [w325] -> w270 mode=indexing
          tunnel: w269 -> [w324] mode=indexing
          tunnel: "%.3f" ("initial string") -> [w323]
          n161 = Format Into String(format string=w323, w324) -> (resulting string=w325:string)  [unwired: 2 in, 1 out]
        }
        n162 = local read "dynamic range (dB)"() -> (w289:dbl[])
        n163 = local read "output power (W)"() -> (w285:dbl[])
        n164 = local read "SFDR (dBc)"() -> (w283:dbl[])
        n165 = local read "gain"() -> (w282:dbl[])
        n166 = for {
          tunnel: [w346] -> w288 mode=indexing
          tunnel: w289 -> [w345] mode=indexing
          tunnel: "%5.1f" ("initial string") -> [w344]
          n167 = Format Into String(format string=w344, w345) -> (resulting string=w346:string)  [unwired: 2 in, 1 out]
        }
        n168 = for {
          tunnel: [w337] -> w268 mode=indexing
          tunnel: w282 -> [w336] mode=indexing
          tunnel: w281 -> [w335]
          n169 = Format Into String(format string=w335, w336) -> (resulting string=w337:string)  [unwired: 2 in, 1 out]
        }
        n170 = for {
          tunnel: [w340] -> w267 mode=indexing
          tunnel: w283 -> [w339] mode=indexing
          tunnel: "%5.1f" ("initial string") -> [w338]
          n171 = Format Into String(format string=w338, w339) -> (resulting string=w340:string)  [unwired: 2 in, 1 out]
        }
        n172 = for {
          tunnel: [w343] -> w266 mode=indexing
          tunnel: w285 -> [w342] mode=indexing
          tunnel: "%.3f" ("initial string") -> [w341]
          n173 = Format Into String(format string=w341, w342) -> (resulting string=w343:string)  [unwired: 2 in, 1 out]
        }
        n174 = Build Array(w261, w278, w275, w272, w270, w287, w295, w292, w288, w268, w267, w266) -> (w265:string[][])
        n175 = Transpose 2D Array(2D array=w265) -> (transposed array=w262:string[][])
        "meas table" <- w262
        n176 = flat-sequence {
          tunnel: [w322] -> w263
          tunnel: w262 -> [_]
          tunnel: w259 -> [w320]
          frame #0 {
            n177 = control-ref of="meas table"() -> (w321:refnum<vi>)
            n178 = call "Autosize Columns (Table).vi"("error in (no error)"=w320, "table"=w321) -> ("error out"=w322:errorcluster)  [unwired: 9 in]
          }
        }
      }
      frame "ShowAnalogUI" {
        n179 = Unbundle By Name(w383) -> ("analog cfg file"=w382:path)
        n180 = Path To String(path=w382) -> (string=w381:string)
        n181 = local write "input configuration file"(w381) -> ()
        n182 = property on="digital channel list" class="Str"("Visible"=FALSE) -> ()  [unwired: 2 in, 2 out]
        n183 = property on="Acquisition channel" class="DAQmxName"("Visible"=TRUE) -> ()  [unwired: 2 in, 2 out]
      }
      frame "ShowDigitalSerialUI" {
        n184 = Unbundle By Name(w389) -> ("digital serial cfg file"=w388:path)
        n185 = Path To String(path=w388) -> (string=w387:string)
        n186 = local write "input configuration file"(w387) -> ()
        n187 = property on="digital channel list" class="Str"("Visible"=TRUE) -> ()  [unwired: 2 in, 2 out]
        n188 = property on="Acquisition channel" class="DAQmxName"("Visible"=FALSE) -> ()  [unwired: 2 in, 2 out]
      }
      frame "Exit" {
        # "This case is triggered to close the User Interface from framework"
        n189 = Flush Queue(queue=w395, error in (no error)=w397) -> (queue out=w394:refnum<queue>, error out=w393:errorcluster)  [unwired: 1 out]
        n190 = Release Queue(queue=w394, force destroy? (F)=TRUE, error in (no error)=w393) -> (error out=w392:errorcluster)  [unwired: 2 out]
      }
      frame "Handle Error" {
      }
    }
  }
